vi "Re-configure Acquisition.vi"(8 "error in (no error)":errorcluster, 10 "Frequency":dbl, 11 "Scope In":refnum<k15>) -> (0 "error out":errorcluster, 3 "Scope out":refnum<k15>)   [LabVIEW 2023, in "Bode Plot - PXI.lvlib"]
doc: "Reconfigures the acquistion, to always acquire ten periods and modifies the vertical range, to use the full dynamic range of the scope"
uses:
  Bode Plot - PXI.lvlib
  <instrlib>/niScope/Controls/niScope vertical coupling.ctl
  <instrlib>/niScope/Controls/niScope array measurement.ctl
  <instrlib>/niScope/Acquire/niScope Multi Read WDT.vi
  <vilib>/measure/mascope.llb/Amplitude and Levels 1 chan.vi
  <vilib>/measure/NI_MAPro.lvlib
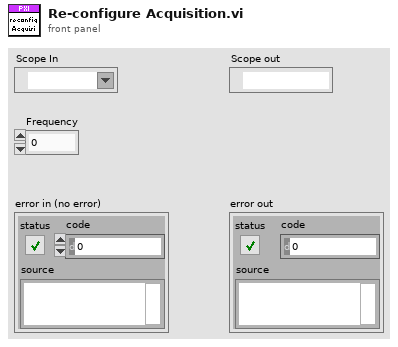
[diagram p1: front panel]
types:
  T1 = typedef "niScope array measurement.ctl" = i32
  T2 = typedef "niScope vertical coupling.ctl" = i32
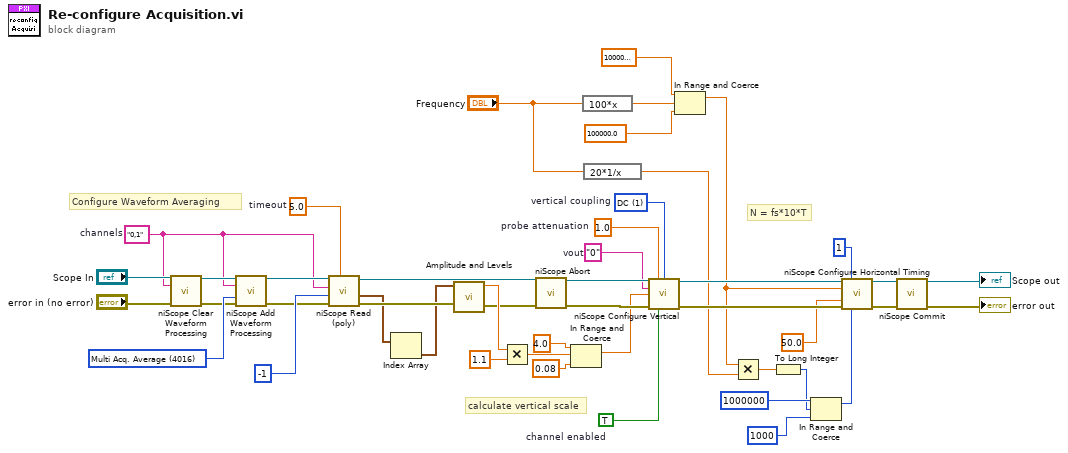
[diagram p0: block diagram]
diagram:
  w11 = T1 4016 items=["None"=4000, "Last Acq. Histogram"=4001, "Multi Acq. Voltage Histogram"=4004, "Multi Acq. Time Histogram"=4005, "Multi Acq. Average"=4016, "Polynomial Interpolation"=4011, "Array Integral"=4006, "Derivative"=4007, "Inverse"=4008, "Multiply Channels"=4012, "Add Channels"=4013, "Subtract Channels"=4014, "Divide Channels"=4015, "Array Offset"=4025, "Array Gain"=4026, "Hanning Window"=4009, "Flat Top Window"=4010, "Hamming Window"=4020, "Triangle Window"=4023, "Blackman Window"=4024, "FIR Windowed Filter"=4021, "Bessel IIR Filter"=4022, "Butterworth IIR Filter"=4017, "Chebyshev IIR Filter"=4018, "FFT Phase Spectrum"=4002, "FFT Amp. Spectrum (Volts RMS)"=4003, "FFT Amp. Spectrum (dB)"=4019] ("array measurement")
  w21 = 5.0  # timeout
  w22 = T2 1 items=["AC", "DC", "Ground"]  # vertical coupling
  w23 = 1.0  # probe attenuation
  w24 = TRUE  # channel enabled
  w26 = "0"  # vout
  w4 = "0,1"  # channels
  # "calculate vertical scale"
  # "Configure Waveform Averaging"
  # "N = fs*10*T"
  n1 = call <instrlib>:"niScope Clear Waveform Processing.vi"("instrument handle"="Scope In", "channels"=w4, "error in"="error in (no error)") -> ("instrument handle out"=w5:refnum<k15>, "error out"=w6:errorcluster)  [unwired: 11 in]
  n2 = call <instrlib>:"niScope Add Waveform Processing.vi"("instrument handle"=w5, "channels"=w4, "array measurement"=w11, "error in"=w6) -> ("instrument handle out"=w10:refnum<k15>, "error out"=w9:errorcluster)  [unwired: 10 in]
  n3 = call-poly <instrlib>:"niScope Read (poly).vi"("timeout"=w21, "error in"=w9, "numSamples"=-1, "channels"=w4, "instrument handle"=w10) -> ("error out"=w40:errorcluster, "wfm"=w27:waveform(dbl)[], "instrument handle out"=w37:refnum<k15>)  [unwired: 3 in, 1 out]
  n4 = Index Array(array=w27) -> (element=w39:waveform(dbl))  [unwired: 1 in]
  n5 = call-poly <vilib>:"Amplitude and Levels.vi"("error in (no error)"=w40, "signal in"=w39) -> ("error out"=w36:errorcluster, "amplitude"=w38:dbl)  [unwired: 6 in, 2 out]
  n6 = Multiply(x=w38, y=1.1) -> (x*y=w3:dbl)
  n7 = call <instrlib>:"niScope Abort.vi"("instrument handle"=w37, "error in"=w36) -> ("instrument handle out"=w35:refnum<k15>, "error out"=w34:errorcluster)  [unwired: 12 in]
  n8 = In Range and Coerce(upper limit=4.0, x=w3, lower limit=0.08) -> (coerced(x)=w25:dbl)  [unwired: 1 out]
  n9 = expression code="100*x"("Frequency") -> (w44:dbl)
  n10 = expression code="20*1/x"("Frequency") -> (w17:dbl)
  n11 = call <instrlib>:"niScope Configure Vertical.vi"("instrument handle"=w35, "probe attenuation"=w23, "vertical coupling"=w22, "channels"=w26, "vertical range"=w25, "error in"=w34, "channel enabled"=w24) -> ("instrument handle out"=w30:refnum<k15>, "error out"=w29:errorcluster)  [unwired: 7 in]
  n12 = In Range and Coerce(upper limit=100000000.0, x=w44, lower limit=100000.0 ("upper limit")) -> (coerced(x)=w1:dbl)  [unwired: 1 out]
  n13 = Multiply(x=w1, y=w17) -> (x*y=w18:dbl)
  n14 = To Long Integer(number=w18) -> (32bit integer=w15:i32)
  n15 = In Range and Coerce(upper limit=1000000, x=w15, lower limit=1000) -> (coerced(x)=w14:i32)  [unwired: 1 out]
  n16 = call <instrlib>:"niScope Configure Horizontal Timing.vi"("instrument handle"=w30, "number of records"=1, "min sample rate"=w1, "reference position"=50.0, "error in"=w29, "min record length"=w14) -> ("instrument handle out"=w31:refnum<k15>, "error out"=w28:errorcluster)  [unwired: 8 in]
  n17 = call <instrlib>:"niScope Commit.vi"("instrument handle"=w31, "error in"=w28) -> ("instrument handle out"=→"Scope out":refnum<k15>, "error out"=→"error out":errorcluster)  [unwired: 12 in]
